vi "Test Rotate.vi"() -> ()   [LabVIEW 2017, in "Image Processing Library.lvlib"]
uses:
  Image Processing Library.lvlib
panel:
  in  "angle [rad]":sgl
  out "Image Rotate":picture
  out "Image In":picture
  out "error out":errorcluster
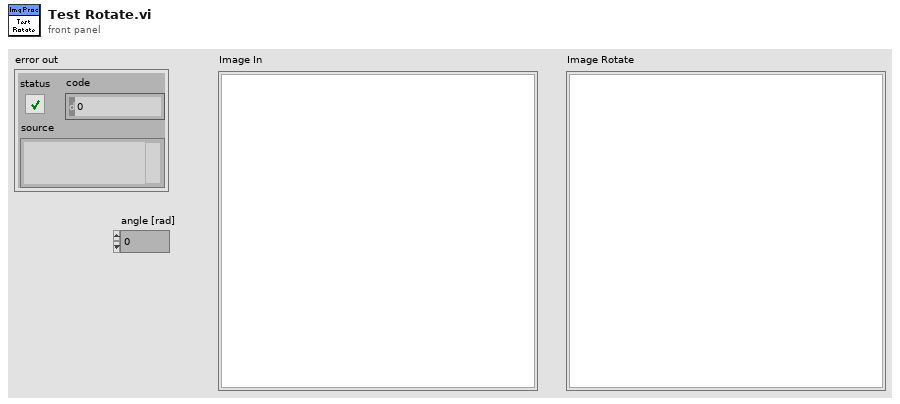
[diagram p1: front panel]
types:
  T1 = typedef "imagedata.ctl" = cluster{"image type":i32, "image depth":i32, "image":u8[], "mask":u8[], "colors":u32[], "Rectangle":cluster{"left":i16, "top":i16, "right":i16, "bottom":i16}}
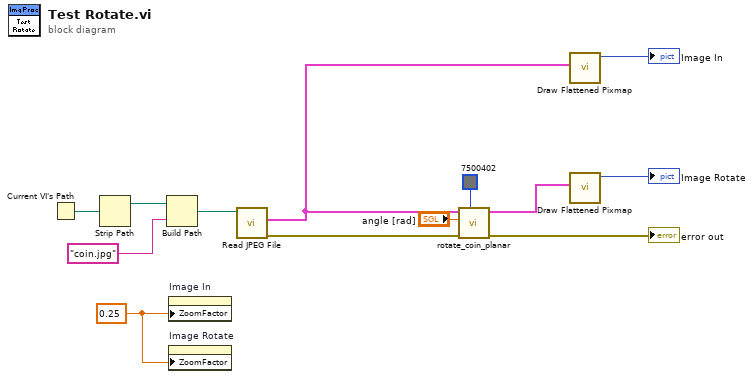
[diagram p0: block diagram]
diagram:
  w6 = sgl 0.25 ("Zoom Factor")
  n1 = Current VI's Path() -> (path=w12:path)
  n2 = Strip Path(path=w12) -> (stripped path=w11:path)  [unwired: 1 out]
  n3 = Build Path(base path=w11, name or relative path="coin.jpg") -> (appended path=w10:path)
  n4 = property on="Image In" class="Pict"("ZoomFactor"=w6) -> ()  [unwired: 2 in, 2 out]
  n5 = property on="Image Rotate" class="Pict"("ZoomFactor"=w6) -> ()  [unwired: 2 in, 2 out]
  n6 = call <vilib>:"Read JPEG File.vi"("path to JPEG file"=w10) -> ("error out"=w9:errorcluster, "image data"=w5:T1)  [unwired: 8 in, 1 out]
  n7 = call "rotate_coin_planar.vi"("pad Color"=u32 7500402, "error in (no error)"=w9, "angle [rad]"="angle [rad]", "image in"=w5) -> ("error out"=→"error out":errorcluster, "image out"=w3:T1)  [unwired: 6 in]
  n8 = call <vilib>:"Draw Flattened Pixmap.vi"("image data"=w5) -> ("new picture"=→"Image In":picture)  [unwired: 8 in]
  n9 = call <vilib>:"Draw Flattened Pixmap.vi"("image data"=w3) -> ("new picture"=→"Image Rotate":picture)  [unwired: 8 in]
